vi "Exo_pair_impair.vi"() -> ()   [LabVIEW 2012]
panel:
  out "Array":dbl[](array[numeric])
  out "Iterations":i32
  in  "N":i32
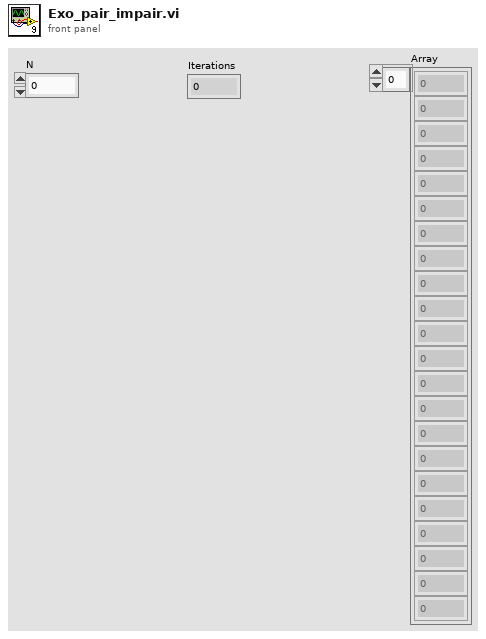
[diagram p1: front panel]
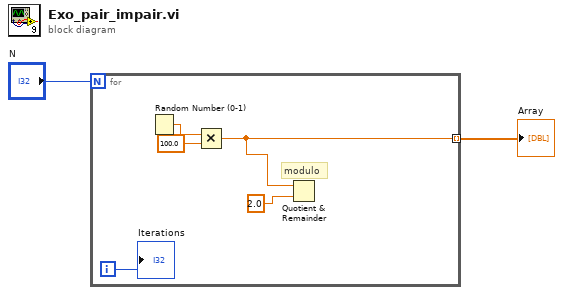
[diagram p0: block diagram]
diagram:
  n1 = for {
    N: "N" -> [_]
    tunnel: [w3] -> w1 mode=indexing
    i -> [w7]
    # "modulo"
    n2 = Random Number (0-1)() -> (number: 0 to 1=w6:dbl)
    n3 = Multiply(x=w6, y=100.0) -> (x*y=w3:dbl)
    n4 = Quotient & Remainder(x=w3, y=2.0) -> ()  [unwired: 2 out]
    "Iterations" <- w7
  }
  "Array" <- w1
